vi "ZM-TST-log.vi"() -> (0 "error out":errorcluster, 3 "Pass":bool)   [LabVIEW 2020, in "ZM-TST-tests.lvlib"]
doc: "T2, test of ZM-CU-log: logs two unique markers and checks that the last two lines of the error log carry them in order, each with an ISO UTC timestamp. Pass = AND of file_ok, order_ok and timestamp_ok. Side effect: two marker lines in the error log."
uses:
  ZM-TST-tests.lvlib
  common/ZM-CU-common_utilities/ZM-CU-common_utilities.lvlib
panel:
  out "timestamp_ok":bool
  out "order_ok":bool
  out "file_ok":bool
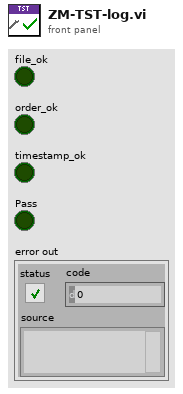
[diagram p1: front panel]
types:
  T1 = enum16{"open", "replace", "create", "open or create", "replace or create", "replace or create with confirmation"}
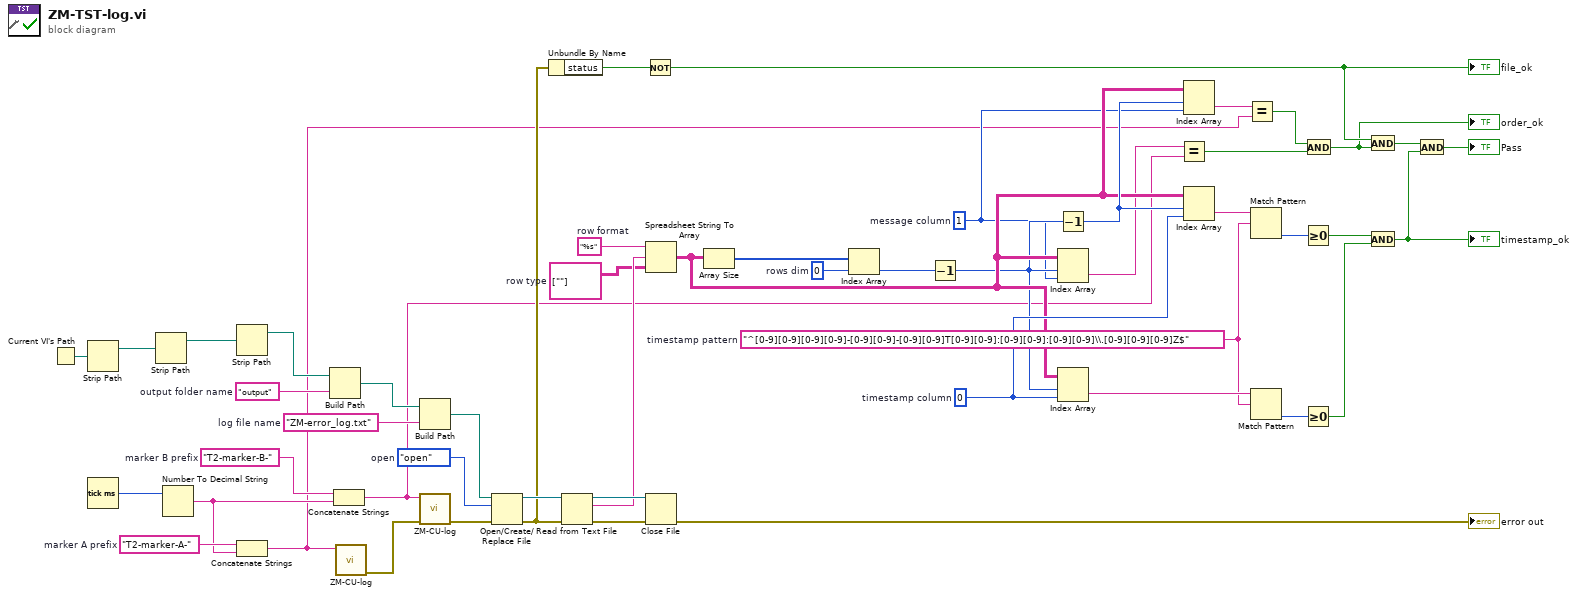
[diagram p0: block diagram]
diagram:
  w10 = "^[0-9][0-9][0-9][0-9]-[0-9][0-9]-[0-9][0-9]T[0-9][0-9]:[0-9][0-9]:[0-9][0-9]\\.[0-9][0-9][0-9]Z$"  # timestamp pattern
  w20 = 1  # message column
  w23 = 0  # timestamp column
  w26 = 0  # rows dim
  w28 = string[][] [[""]]  # row type
  w30 = "%s"  # row format
  w37 = T1."open"  # open
  w39 = "ZM-error_log.txt"  # log file name
  w41 = "output"  # output folder name
  w48 = "T2-marker-B-"  # marker B prefix
  w49 = "T2-marker-A-"  # marker A prefix
  n1 = Current VI's Path() -> (path=w45:path)
  n2 = Strip Path(path=w45) -> (stripped path=w44:path)  [unwired: 1 out]
  n3 = Tick Count (ms)() -> (millisecond timer value=w50:u32)
  n4 = Strip Path(path=w44) -> (stripped path=w43:path)  [unwired: 1 out]
  n5 = Number To Decimal String(number=w50) -> (decimal integer string=w47:string)  [unwired: 1 in]
  n6 = Strip Path(path=w43) -> (stripped path=w42:path)  [unwired: 1 out]
  n7 = Concatenate Strings(w49, w47) -> (w18:string)
  n8 = Build Path(base path=w42, name or relative path=w41) -> (appended path=w40:path)
  n9 = Concatenate Strings(w48, w47) -> (w16:string)
  n10 = call "ZM-CU-log.vi"("message"=w18) -> ("error out"=w46:errorcluster)  [unwired: 10 in]
  n11 = Build Path(base path=w40, name or relative path=w39) -> (appended path=w38:path)
  n12 = call "ZM-CU-log.vi"("error in"=w46, "message"=w16) -> ("error out"=w36:errorcluster)  [unwired: 9 in]
  n13 = Open/Create/Replace File(file path (use dialog)=w38, error in=w36, operation (0:open)=w37) -> (refnum out=w34:refnum<file>, error out=w33:errorcluster)  [unwired: 3 in, 1 out]
  n14 = Unbundle By Name(w33) -> ("status"=w35:bool)
  n15 = Read from Text File(file (use dialog)=w34, error in=w33) -> (refnum out=w32:refnum<file>, text=w29:string, error out=w31:errorcluster)  [unwired: 2 in, 1 out]
  n16 = Not(x=w35) -> (.not. x?=w5:bool)
  "file_ok" <- w5
  n17 = Spreadsheet String To Array(format string=w30, spreadsheet string=w29, array type (2D Dbl)=w28) -> (array=w22:string[][])  [unwired: 1 in]
  n18 = Close File(refnum=w32, error in=w31) -> (error out=→"error out":errorcluster)  [unwired: 1 out]
  n19 = Array Size(array=w22) -> (size(s)=w27:i32[])
  n20 = Index Array(array=w27, index=w26) -> (element=w25:i32)
  n21 = Decrement(x=w25) -> (x-1=w21:i32)
  n22 = Decrement(x=w21) -> (x-1=w24:i32)
  n23 = Index Array(array=w22, index (row)=w21, index (col)=w20) -> (element=w17:string)
  n24 = Index Array(array=w22, index (row)=w21, index (col)=w23) -> (element=w11:string)
  n25 = Equal?(x=w17, y=w16) -> (x = y?=w14:bool)
  n26 = Index Array(array=w22, index (row)=w24, index (col)=w20) -> (element=w19:string)
  n27 = Index Array(array=w22, index (row)=w24, index (col)=w23) -> (element=w13:string)
  n28 = Equal?(x=w19, y=w18) -> (x = y?=w15:bool)
  n29 = Match Pattern(string=w13, regular expression=w10) -> (offset past match=w12:i32)  [unwired: 1 in, 3 out]
  n30 = Match Pattern(string=w11, regular expression=w10) -> (offset past match=w9:i32)  [unwired: 1 in, 3 out]
  n31 = Greater Or Equal To 0?(x=w12) -> (x >= 0?=w8:bool)
  n32 = Greater Or Equal To 0?(x=w9) -> (x >= 0?=w7:bool)
  n33 = And(x=w15, y=w14) -> (x .and. y?=w4:bool)
  "order_ok" <- w4
  n34 = And(x=w5, y=w4) -> (x .and. y?=w6:bool)
  n35 = And(x=w8, y=w7) -> (x .and. y?=w3:bool)
  "timestamp_ok" <- w3
  n36 = And(x=w6, y=w3) -> (x .and. y?=→"Pass":bool)
